vi "Create.vi"(4 "Event Filter":refnum<class "WebView2 Event Filter Interface.lvclass">, 6 "Register Events (F)":bool, 8 "error in (no error)":errorcluster, 10 "WebView2 Control":refnum<k24>, 11 "Type":refnum<class "WebView2 Control.lvclass">) -> (0 "error out":errorcluster, 3 "WebView2 Control out":refnum<class "WebView2 Control.lvclass">)   [LabVIEW 2020, in "WebView2.lvlib" / "WebView2 Control.lvclass"]
uses:
  WebView2 Control.lvclass
  E:/Labview/LV 2023/PPL/PPL Builder/Libs/LV-WebView2/Source/Libs/Microsoft.Web.WebView2.WinForms.dll
  Libs/Microsoft.Web.WebView2.WinForms.dll
  WebView2 Event Filter Interface/WebView2 Event Filter Interface.lvclass
  WebView2 Control.lvclass/WebView2 Control.ctl
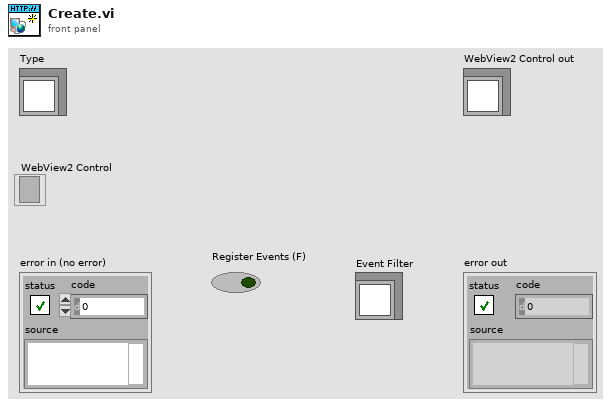
[diagram p1: front panel]
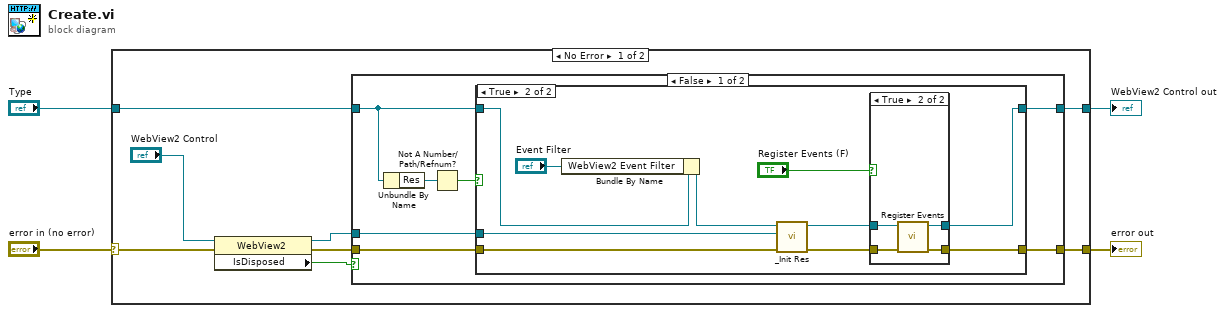
[diagram p0: block diagram]
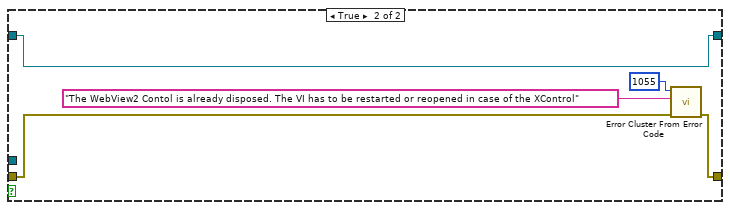
[diagram p4: hidden frame]
diagram:
  n1 = case shown="No Error" "error in (no error)" {
    selector: "error in (no error)" -> [w10 w44]
    tunnel: [w5 w44] -> w3
    tunnel: [w12 w43] -> w1
    tunnel: "Type" -> [w11 w43]
    frame No Error {
      n2 = property class="WebView2"(reference="WebView2 Control", error in=w10) -> (reference out=w8:refnum<k24>, error out=w6:errorcluster, "IsDisposed"=w7:bool)
      n3 = case shown="False" w7 {
        tunnel: [w19 w42] -> w12
        tunnel: w11 -> [w17 w42]
        tunnel: w8 -> [w18 _]
        tunnel: w6 -> [w14 w39]
        tunnel: [w13 w38] -> w5
        frame False {
          n4 = Unbundle By Name(w17) -> ("Res"=w16:refnum<data-value>)
          n5 = Not A Number/Path/Refnum?(number/path/refnum=w16) -> (NaN/Path/Refnum?=w15:bool)
          n6 = case shown="True" w15 {
            tunnel: [w21 w23] -> w19
            tunnel: w18 -> [_ w31]
            tunnel: w17 -> [w21 w30]
            tunnel: w14 -> [w20 w29]
            tunnel: [w20 w25] -> w13
            frame False {
              # "already init'ed"
            }
            frame True {
              n7 = Bundle By Name(cluster=w30, "WebView2 Event Filter"="Event Filter") -> (w27:refnum<class "WebView2 Control.lvclass">)
              n8 = call "_Init Res.vi"("error in (no error)"=w29, "WebView2 Control"=w31, "WebView2 Control in"=w27) -> ("error out"=w28:errorcluster, "WebView2 Control out"=w24:refnum<class "WebView2 Control.lvclass">)  [unwired: 7 in]
              n9 = case shown="True" "Register Events (F)" {
                tunnel: w28 -> [w32 w37]
                tunnel: [w32 w36] -> w25
                tunnel: w24 -> [w33 w35]
                tunnel: [w33 w34] -> w23
                frame False {
                }
                frame True {
                  n10 = call "Register Events.vi"("error in (no error)"=w37, "WebView2 Control in"=w35) -> ("error out"=w36:errorcluster, "WebView2 Control out"=w34:refnum<class "WebView2 Control.lvclass">)  [unwired: 7 in, 1 out]
                }
              }
            }
          }
        }
        frame True {
          n11 = call <vilib>:"Error Cluster From Error Code.vi"("error in (no error)"=w39, "error message (\"\")"="The WebView2 Contol is already disposed. The VI has to be restarted or reopened in case of the XControl" ("error message (\"\")"), "error code (0)"=1055) -> ("error out"=w38:errorcluster)  [unwired: 6 in]
        }
      }
    }
    frame Error {
    }
  }
  "error out" <- w3
  "WebView2 Control out" <- w1
